vi "OwnMethod20261013_RelinkSubVI.vi"() -> ()   [LabVIEW 2024]
panel:
  out "error out":errorcluster caption="错误输出"
  in  "Path":path
  out "path error out":errorcluster caption="错误输出"
  out "vi_path":path
  in  "subvi_id":u32
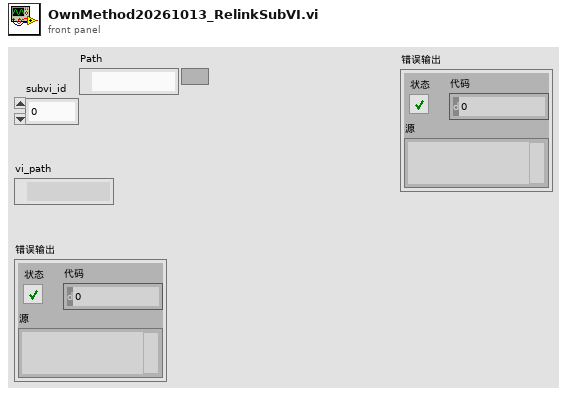
[diagram p1: front panel]
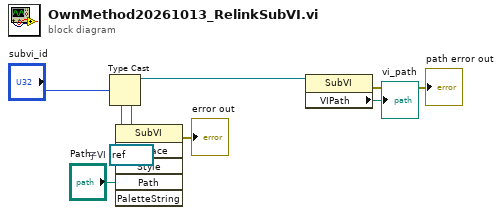
[diagram p0: block diagram]
diagram:
  w6 = refnum<vi> refnum  # 子VI
  n1 = Type Cast ("强制类型转换")(type=w6, x="subvi_id") -> (*(type *) &x=w5:refnum<vi>)
  n2 = invoke class="SubVI" method="Replace"(reference=w5, "Path"="Path") -> (error out=→"error out":errorcluster)  [unwired: 4 in, 5 out]
  n3 = property on="属性节点" class="SubVI"(reference=w5) -> (error out=→"path error out":errorcluster, "VIPath"=→"vi_path":path)  [unwired: 1 in, 1 out]
